vi "Load Plot.vi"(8 "error in (no error)":errorcluster, 10 "Plot Index":i32, 11 "Data Viewer in":refnum<class "Data Viewer.lvclass">) -> (0 "error out":errorcluster, 1 "Cancel?":bool, 2 "Plot Name":string, 3 "Data Viewer out":refnum<class "Data Viewer.lvclass">)   [LabVIEW 2020, in "Data Viewer.lvlib" / "Data Viewer.lvclass"]
uses:
  Data Viewer.lvclass
  File Type--enum.ctl
  Data Serie--cluster.ctl
  Data Viewer.lvclass/Data Viewer.ctl
  Data Viewer.lvlib
panel:
  out "Row":i32
  out "In Range?":bool
  in  "Tab Control":enum32{"Page 2"}(tab)
  in  "ReSample":bool
  in  "重采样率[Hz]":dbl format="%.3f"
  out "结束时间":timestamp format="%<%x %.3X>T"
  out "开始时间":timestamp format="%<%x %.3X>T"
  out "Δt[S]":dbl format="%.3f"
  out "数据量":i32
  out "采样率[Hz]":dbl format="%.3f"
  in  "文件参数":T1={"分隔符"=enum."逗号", "数据首列"=2, "数据首行"=5, "单位行"=4, "名称行"=4, "时间列"=1}
  in  "数据列表":i32(listbox)
  in  "File Type":T2 caption="数据类型"
  out "File Path":path caption="文件路径"
  in  "Open File":bool
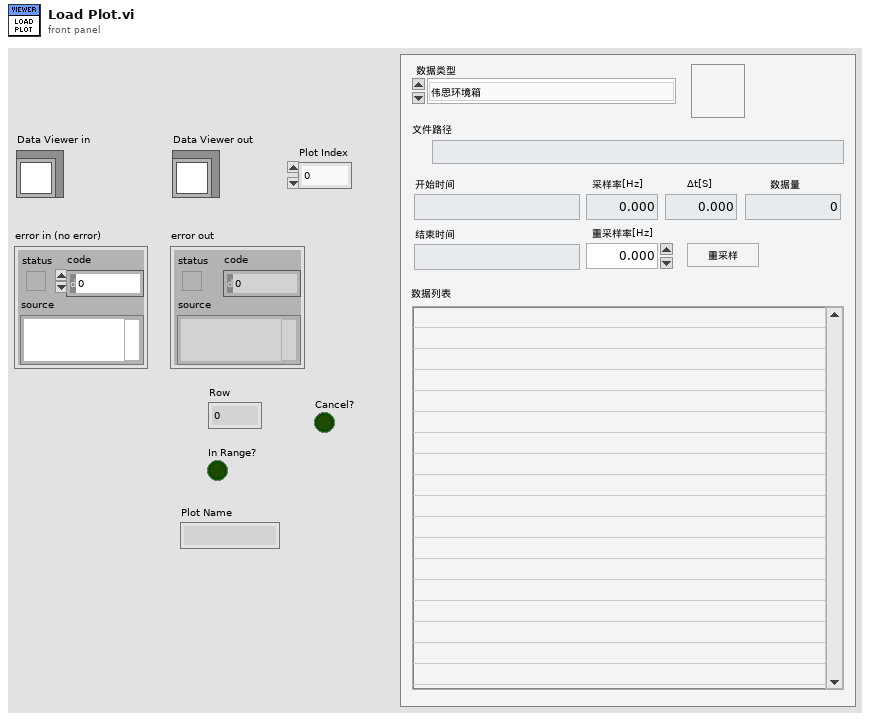
[diagram p1: front panel]
types:
  T1 = cluster{"分隔符":enum16{"逗号", "制表符"}, "数据首列":i32, "数据首行":i32, "单位行":i32, "名称行":i32, "时间列":i32}
  T2 = typedef "Data Viewer.lvlib/File Type--enum.ctl" = enum16{"伟思环境箱", "增达环境箱", "广五所环境箱", "无纸记录仪", "帕捷SA00339", "记录仪840", "记录仪8400", "记录仪MR888", "*.csv"}
  T3 = enum32{"Invalid", "Standard", "Closed", "Hidden", "Minimized", "Maximized"}
  T4 = typedef "Data Viewer.lvlib/Data Serie--cluster.ctl" = cluster{"Name":string, "Unit":string, "Sample Rate[Hz]":dbl, "Delta t[S]":dbl, "t0":timestamp, "Length":i32, "Time":timestamp[], "Value":dbl[]}
  T5 = typedef "LVPoint32TypeDef.ctl" = cluster{"Horizontal":i32, "Vertical":i32}
  T6 = typedef "Data Viewer.lvlib/Data Viewer.lvclass/Plot Property--cluster.ctl" = cluster{"Name":string, "Visible":bool, "Color":u32, "Scale Index":i32, "Show Peak Line":bool}
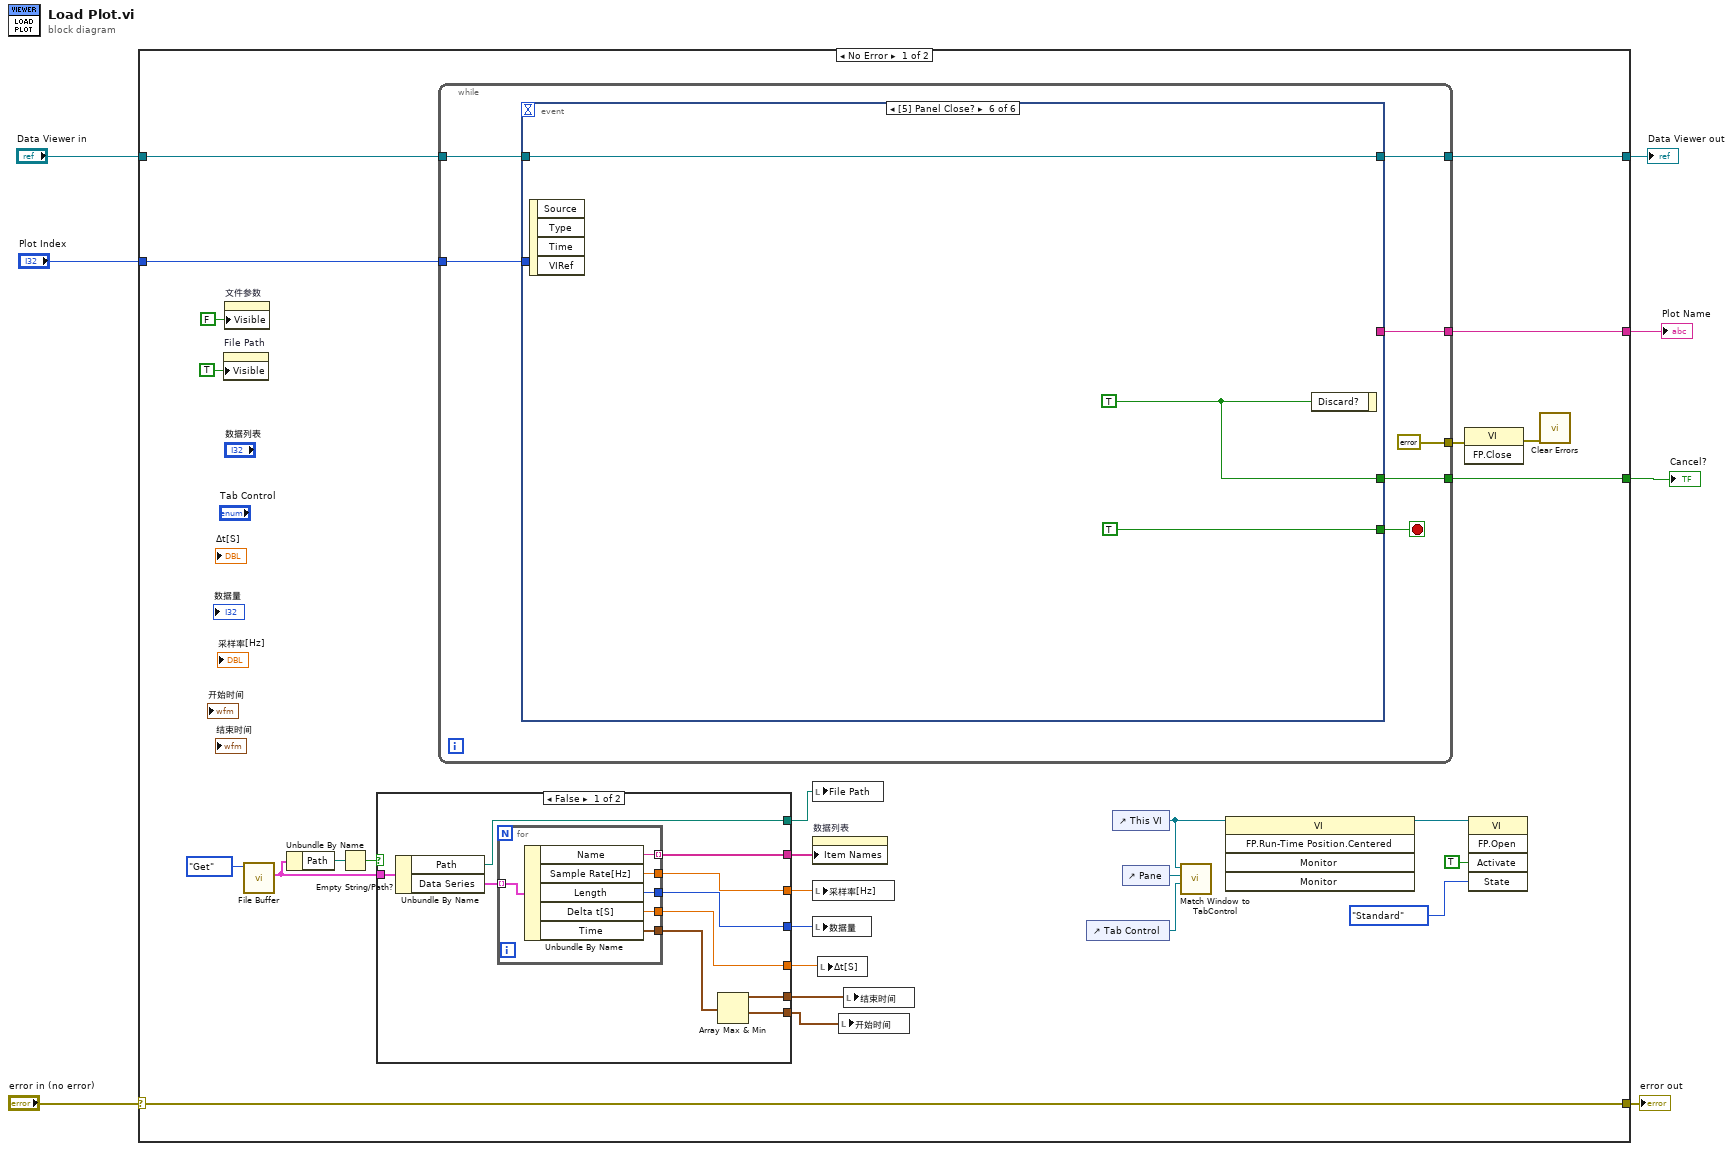
[diagram p0: block diagram]
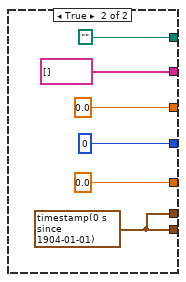
[diagram p2: hidden frame]
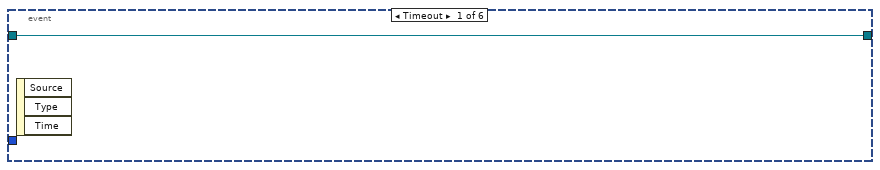
[diagram p3: hidden frame]
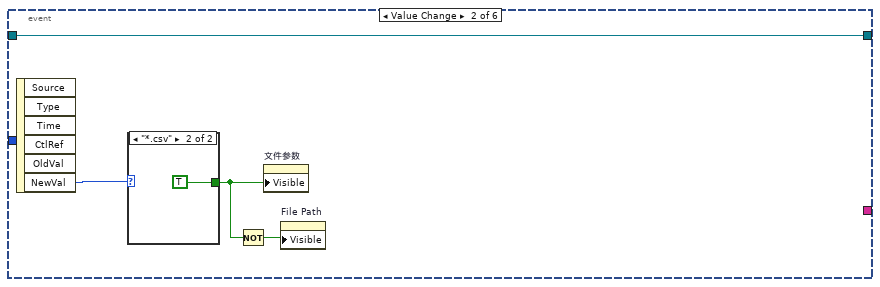
[diagram p4: hidden frame]
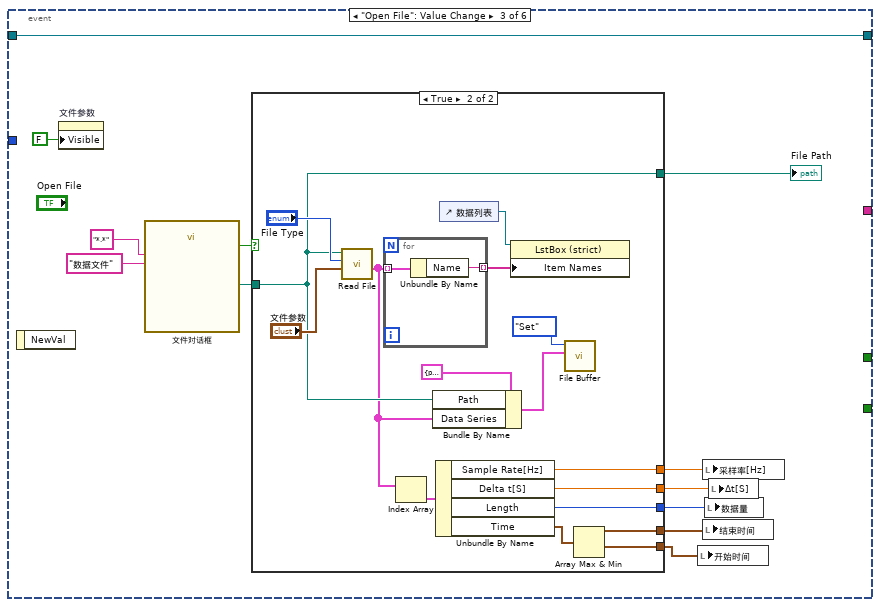
[diagram p6: hidden frame]
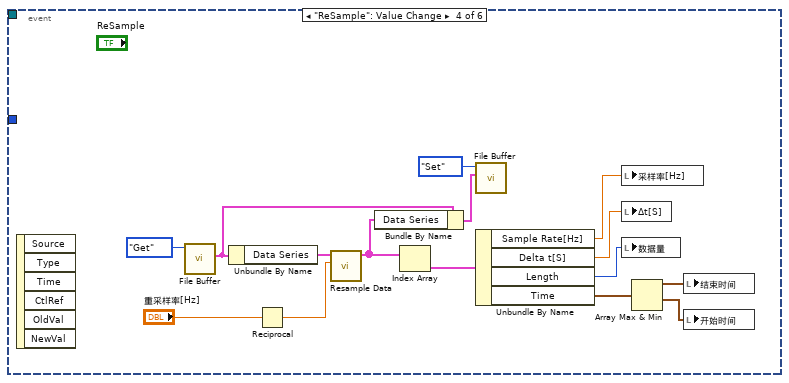
[diagram p8: hidden frame]
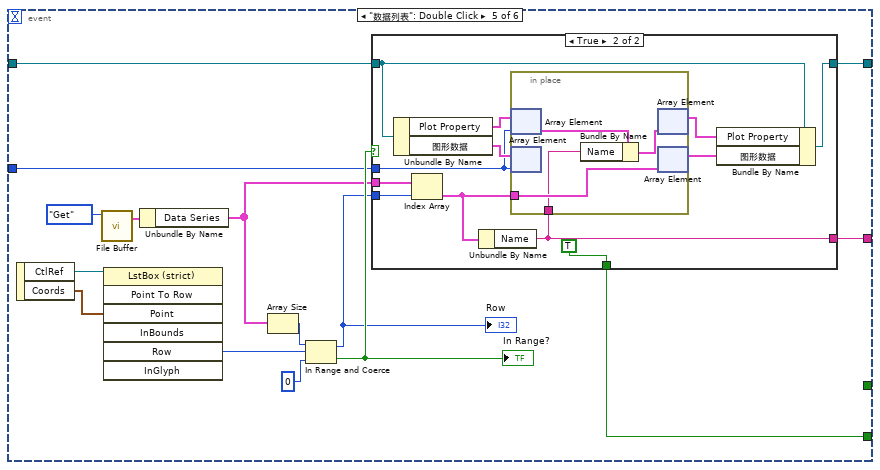
[diagram p9: hidden frame]
diagram:
  n1 = case shown="No Error" "error in (no error)" {
    selector: "error in (no error)" -> [w34 w151]
    tunnel: [w34 w151] -> w6
    tunnel: [w25 w150] -> w4
    tunnel: "Data Viewer in" -> [w26 w150]
    tunnel: "Plot Index" -> [w24 _]
    tunnel: [w23 _] -> w2
    tunnel: [w8 _] -> w1
    frame No Error {
      n2 = property on="File Path" class="Path"("Visible"=TRUE) -> ()  [unwired: 2 in, 2 out]
      n3 = property on="文件参数" class="Clust (strict)"("Visible"=FALSE) -> ()  [unwired: 2 in, 2 out]
      n4 = call "File Buffer.vi"("Operation"=enum16{"Get", "Set"}."Get") -> ("File Buffer Out"=w16:cluster{"Path":path, "Data Series":T4[]})  [unwired: 10 in]
      n5 = Unbundle By Name(w16) -> ("Path"=w19:path)
      n6 = Empty String/Path?(string/path=w19) -> (empty?=w18:bool)
      n7 = case shown="False" w18 {
        tunnel: [w43 path ""] -> w17
        tunnel: [w41 string[] [] ("Item Names")] -> w15
        tunnel: w16 -> [w44 _]
        tunnel: [w40 0.0 ("Sample Rate[Hz]")] -> w14
        tunnel: [w39 0 ("Length")] -> w13
        tunnel: [w38 0.0 ("Δt[S]")] -> w12
        tunnel: [w36 w51] -> w9
        tunnel: [w35 w51] -> w10
        frame False {
          n8 = Unbundle By Name(w44) -> ("Path"=w43:path, "Data Series"=w42:T4[])
          n9 = for {
            tunnel: w42 -> [w50] mode=indexing
            tunnel: [w49] -> w41 mode=indexing
            tunnel: [w48] -> w40
            tunnel: [w47] -> w39
            tunnel: [w46] -> w38
            tunnel: [w45] -> w37
            n10 = Unbundle By Name(w50) -> ("Name"=w49:string, "Sample Rate[Hz]"=w48:dbl, "Length"=w47:i32, "Delta t[S]"=w46:dbl, "Time"=w45:timestamp[])
          }
          n11 = Array Max & Min(array=w37) -> (max value=w35:timestamp, min value=w36:timestamp)  [unwired: 2 out]
        }
        frame True {
          w51 = timestamp(0 s since 1904-01-01)
        }
      }
      n12 = while {
        tunnel: w26 -> [w62]
        tunnel: [w61] -> w25
        tunnel: w24 -> [w60]
        tunnel: [w59] -> w23
        tunnel: [errorcluster {"status"=FALSE, "code"=0, "source"=""} ("error in (no error)")] -> w22
        tunnel: [w57] -> w8
        stop <- w63 stop-if-true
        n13 = event shown="[5] Panel Close?" {
          selector: _ -> [_ _ _ _ _ _]
          dyn-events: _ -> [_ _ _ _ _ _]
          timeout: _ -> [_ _ _ _ _ _]
          tunnel: [_ _ _ _ w118 TRUE] -> w63
          tunnel: [w64 w67 w76 _ w124 w148] -> w61
          tunnel: w62 -> [w64 w67 w76 _ w123 w148]
          tunnel: w60 -> [_ _ _ _ w121 _]
          tunnel: [_ _ _ _ w119 _] -> w59
          tunnel: [_ _ _ _ _ w147] -> w57
          event Timeout {
            n14 = event-data() -> ()  [unwired: 1 in, 3 out]
          }
          event Value Change {
            n15 = event-data() -> ("NewVal"=w68:T2)  [unwired: 1 in, 5 out]
            n16 = case shown="\"*.csv\"" w68 {
              tunnel: [_ TRUE] -> w65
              frame "伟思环境箱", Default {
              }
              frame "*.csv" {
              }
            }
            n17 = Not(x=w65) -> (.not. x?=w66:bool)
            n18 = property on="文件参数" class="Clust (strict)"("Visible"=w65) -> ()  [unwired: 2 in, 2 out]
            n19 = property on="File Path" class="Path"("Visible"=w66) -> ()  [unwired: 2 in, 2 out]
          }
          event "Open File": Value Change {
            n20 = event-data() -> ()  [unwired: 1 in, 1 out]
            n21 = property on="文件参数" class="Clust (strict)"("Visible"=FALSE) -> ()  [unwired: 2 in, 2 out]
            n22 = call "文件对话框"("pattern (all files)"="*.*", "pattern label"="数据文件") -> ("selected path"=w78:path, "exists"=w79:bool)  [unwired: 10 in, 2 out]
            n23 = case shown="True" w79 {
              tunnel: w78 -> [_ w93]
              tunnel: [_ w93] -> w75
              tunnel: [_ w87] -> w74
              tunnel: [_ w86] -> w73
              tunnel: [_ w85] -> w72
              tunnel: [_ w83] -> w70
              tunnel: [_ w82] -> w71
              frame False {
              }
              frame True {
                n24 = call "Read File.vi"("文件参数"="文件参数", "File Type"="File Type", "Path"=w93) -> ("Data Series"=w89:T4[])  [unwired: 8 in]
                n25 = for {
                  tunnel: w89 -> [w99] mode=indexing
                  tunnel: [w98] -> w94 mode=indexing
                  n26 = Unbundle By Name(w99) -> ("Name"=w98:string)
                }
                n27 = Index Array(array=w89) -> (element=w88:T4)  [unwired: 1 in]
                n28 = Bundle By Name(cluster=cluster{"Path":path, "Data Series":T4[]} {"Path"=path "", "Data Series"=[]}, "Path"=w93, "Data Series"=w89) -> (w92:cluster{"Path":path, "Data Series":T4[]})
                n29 = Unbundle By Name(w88) -> ("Sample Rate[Hz]"=w87:dbl, "Delta t[S]"=w86:dbl, "Length"=w85:i32, "Time"=w84:timestamp[])
                n30 = control-ref of="数据列表"() -> (w95:refnum<vi>)
                n31 = property class="LstBox (strict)"(reference=w95, "Item Names"=w94) -> ()  [unwired: 1 in, 2 out]
                n32 = call "File Buffer.vi"("File Buffer In"=w92, "Operation"=enum16{"Get", "Set"}."Set") -> ()  [unwired: 9 in, 1 out]
                n33 = Array Max & Min(array=w84) -> (max value=w83:timestamp, min value=w82:timestamp)  [unwired: 2 out]
              }
            }
            "File Path" <- w75
            n34 = local write "开始时间"(w71) -> ()
            n35 = local write "采样率[Hz]"(w74) -> ()
            n36 = local write "结束时间"(w70) -> ()
            n37 = local write "数据量"(w72) -> ()
            n38 = local write "Δt[S]"(w73) -> ()
          }
          event "ReSample": Value Change {
            n39 = event-data() -> ()  [unwired: 1 in, 6 out]
            n40 = call "File Buffer.vi"("Operation"=enum16{"Get", "Set"}."Get") -> ("File Buffer Out"=w110:cluster{"Path":path, "Data Series":T4[]})  [unwired: 10 in]
            n41 = Unbundle By Name(w110) -> ("Data Series"=w113:T4[])
            n42 = Reciprocal(x="重采样率[Hz]") -> (1/x=w111:dbl)
            n43 = call "Resample Data.vi"("dt"=w111, "Data Series In"=w113) -> ("Data Series Out"=w109:T4[])  [unwired: 9 in]
            n44 = Bundle By Name(cluster=w110, "Data Series"=w109) -> (w101:cluster{"Path":path, "Data Series":T4[]})
            n45 = Index Array(array=w109) -> (element=w108:T4)  [unwired: 1 in]
            n46 = call "File Buffer.vi"("File Buffer In"=w101, "Operation"=enum16{"Get", "Set"}."Set") -> ()  [unwired: 9 in, 1 out]
            n47 = Unbundle By Name(w108) -> ("Sample Rate[Hz]"=w107:dbl, "Delta t[S]"=w106:dbl, "Length"=w105:i32, "Time"=w104:timestamp[])
            n48 = local write "采样率[Hz]"(w107) -> ()
            n49 = local write "Δt[S]"(w106) -> ()
            n50 = local write "数据量"(w105) -> ()
            n51 = Array Max & Min(array=w104) -> (max value=w103:timestamp, min value=w102:timestamp)  [unwired: 2 out]
            n52 = local write "结束时间"(w103) -> ()
            n53 = local write "开始时间"(w102) -> ()
          }
          event "数据列表": Double Click {
            n54 = event-data() -> ("CtlRef"=w129:refnum<vi>, "Coords"=w128:T5)  [unwired: 1 in]
            n55 = call "File Buffer.vi"("Operation"=enum16{"Get", "Set"}."Get") -> ("File Buffer Out"=w116:cluster{"Path":path, "Data Series":T4[]})  [unwired: 10 in]
            n56 = invoke class="LstBox (strict)" method="Point To Row"(reference=w129, "Point"=w128) -> ("Row"=w127:i32)  [unwired: 5 in, 6 out]
            n57 = Unbundle By Name(w116) -> ("Data Series"=w117:T4[])
            n58 = Array Size(array=w117) -> (size(s)=w125:i32)
            n59 = In Range and Coerce(upper limit=w125, x=w127, lower limit=0) -> (coerced(x)=w120:i32, In Range?=w122:bool)
            "Row" <- w120
            "In Range?" <- w122
            n60 = case shown="True" w122 {
              tunnel: [w130 w138] -> w124
              tunnel: w123 -> [w130 w142]
              tunnel: w117 -> [_ w140]
              tunnel: w121 -> [_ w131]
              tunnel: w120 -> [_ w139]
              tunnel: [_ w132] -> w119
              tunnel: [_ TRUE] -> w118
              frame False {
              }
              frame True {
                n61 = Unbundle By Name(w142) -> ("Plot Property"=w134:T6[], "图形数据"=w141:T4[])
                n62 = Index Array(array=w140, index=w139) -> (element=w136:T4)
                n63 = Unbundle By Name(w136) -> ("Name"=w132:string)
                n64 = in-place {
                  in-place-border: w136 -> [w146]
                  in-place-border: w132 -> [w144]
                  n65 = in-place-array #1(w134, w131) -> (w145:T6)
                  n66 = in-place-array #2(w141, w131) -> ()  [unwired: 1 out]
                  n67 = Bundle By Name(cluster=w145, "Name"=w144) -> (w143:T6)
                  n68 = in-place-array #1(w143) -> (w133:T6[])  [unwired: 1 out]
                  n69 = in-place-array #2(w146) -> (w137:T4[])  [unwired: 1 out]
                }
                n70 = Bundle By Name(cluster=w142, "Plot Property"=w133, "图形数据"=w137) -> (w138:refnum<class "Data Viewer.lvclass">)
              }
            }
          }
          event Panel Close? {
            w147 = TRUE ("Discard?")
            n71 = event-data() -> ()  [unwired: 1 in, 4 out]
            n72 = event-data("Discard?"=w147) -> ()  [unwired: 1 in, 1 out]
          }
        }
      }
      n73 = local write "File Path"(w17) -> ()
      n74 = property on="数据列表" class="LstBox (strict)"("Item Names"=w15) -> ()  [unwired: 2 in, 2 out]
      n75 = local write "采样率[Hz]"(w14) -> ()
      n76 = local write "数据量"(w13) -> ()
      n77 = local write "Δt[S]"(w12) -> ()
      n78 = local write "开始时间"(w9) -> ()
      n79 = local write "结束时间"(w10) -> ()
      n80 = control-ref of="Tab Control"() -> (w33:refnum<vi>)
      n81 = control-ref of="This VI"() -> (w30:refnum<vi>)
      n82 = control-ref of="Pane"() -> (w32:refnum<vi>)
      n83 = call "Match Window to TabControl.vi"("Tab Control"=w33, "Pane"=w32, "VI in"=w30) -> ()  [unwired: 9 in]
      n84 = invoke class="VI" method="FP.Run-Time Position.Centered"(reference=w30) -> (reference out=w29:refnum<vi>)  [unwired: 4 in, 4 out]
      n85 = invoke class="VI" method="FP.Close"(error in=w22) -> (error out=w21:errorcluster)  [unwired: 2 in, 2 out]
      n86 = invoke class="VI" method="FP.Open"(reference=w29, "Activate"=TRUE ("Activate?"), "State"=T3."Standard") -> ()  [unwired: 2 in, 5 out]
      n87 = call <vilib>:"Clear Errors.vi"("error in (no error)"=w21) -> ()  [unwired: 5 in, 2 out]
    }
    frame Error {
    }
  }
  "error out" <- w6
  "Data Viewer out" <- w4
  "Plot Name" <- w2
  "Cancel?" <- w1
